vi "GpuMat RowRange.vi"(8 "error in (no error)":errorcluster, 9 "EndRow":i32, 10 "StartRow":i32, 11 "Src in":refnum<class "GpuMat.lvclass">) -> (0 "error out":errorcluster, 2 "Clone out":refnum<class "GpuMat.lvclass">, 3 "Src out":refnum<class "GpuMat.lvclass">)   [LabVIEW 2020, in "OpenLvVision_OpenCv.lvlib" / "Cuda.lvlib" / "GpuMat.lvclass"]
doc: "returns a new GpuMat header for the specified row span"
uses:
  GpuMat.lvclass
  C:/Users/lukas/Documents/OpenLvVision_OpenCv/SourceCode/LabView/OpenLvVision_OpenCv/_LvHelpers/EdvrObject/EdvrObject.lvclass
  _LvHelpers/EdvrObject/EdvrObject.lvclass/EdvrObject.ctl
  _LvHelpers/EdvrObject/TypeDef/Edvr.ctl
  OpenLvVision_OpenCv.lvlib
  <vilib>/Utility/error.llb/Error Cluster From Error Code.vi
  <vilib>/ErrorRing/Error Ring.xnode
  _LvHelpers/EdvrObject/EdvrObject.lvclass
  Dlls/OlvOpenCvWrapper.dll
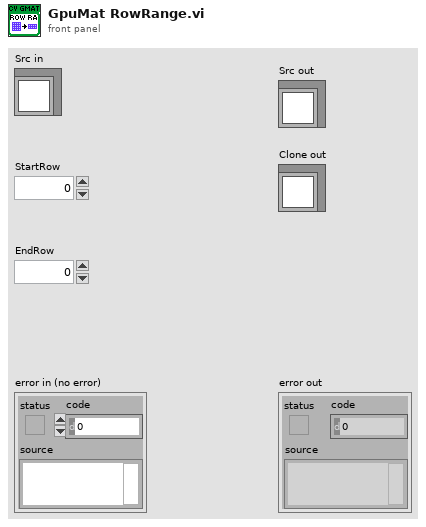
[diagram p1: front panel]
types:
  T1 = typedef "OpenLvVision_OpenCv.lvlib/EdvrObject.lvclass/Edvr.ctl" = refnum<data-value>
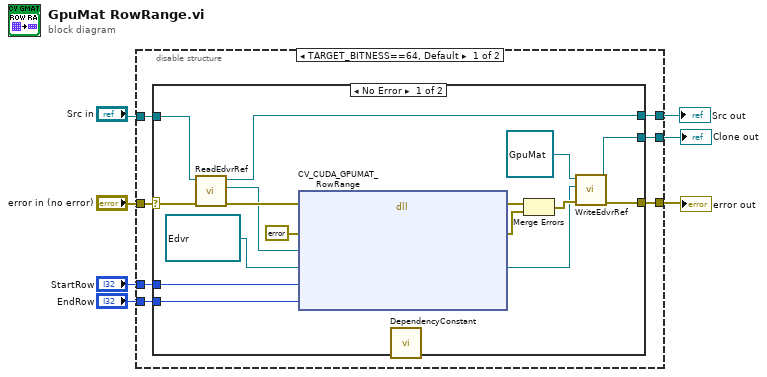
[diagram p0: block diagram]
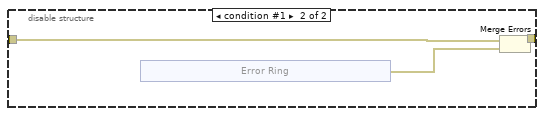
[diagram p3: hidden frame]
diagram:
  n1 = disable-structure shown="TARGET_BITNESS==64, Default" {
    disable-tunnel: "error in (no error)" -> [w14 w34]
    disable-tunnel: [w13 w35] -> w7
    disable-tunnel: "Src in" -> [w12 _]
    disable-tunnel: [w11 _] -> w4
    disable-tunnel: [w10 _] -> w3
    disable-tunnel: "StartRow" -> [w9 _]
    disable-tunnel: "EndRow" -> [w8 _]
    frame condition #0 (active) {
      n2 = case shown="No Error" w14 {
        selector: w14 -> [w23 w32]
        tunnel: [w21 w32] -> w13
        tunnel: w12 -> [w25 w31]
        tunnel: [w24 w31] -> w11
        tunnel: [w19 _] -> w10
        tunnel: w9 -> [w16 _]
        tunnel: w8 -> [w15 _]
        frame No Error {
          n3 = call "ReadEdvrRef.vi"("error in (no error)"=w23, "EdvrObject in"=w25) -> ("error out"=w27:errorcluster, "Edvr"=w26:T1, "EdvrObject out"=w24:refnum<class "GpuMat.lvclass">)  [unwired: 7 in]
          n4 = dll-call lib="C:/Users/lukas/Documents/OpenLvVision_OpenCv/SourceCode/LabView/OpenLvVision_OpenCv/Dlls/OlvOpenCvWrapper.dll" fn="CV_CUDA_GPUMAT_RowRange"(error in=w27, "Error"=errorcluster {"status"=FALSE, "code"=0, "source"=""} ("error out"), "srcRef"=w26, "dstRef"=T1 refnum ("Edvr"), "startCol"=w16, "endCol"=w15) -> (error out=w30:errorcluster, "Error"=w29:errorcluster, "dstRef"=w18:T1)  [unwired: 6 in, 1 out]
          n5 = call "DependencyConstant.vi"() -> ()  [unwired: 12 in]
          n6 = Merge Errors(w30, w29) -> (w22:errorcluster)
          n7 = call "WriteEdvrRef.vi"("error in (no error)"=w22, "Edvr"=w18, "EdvrObject in"=refnum<class "GpuMat.lvclass"> refnum ("Dst out")) -> ("error out"=w21:errorcluster, "EdvrObject out"=w19:refnum<class "GpuMat.lvclass">)  [unwired: 7 in]
        }
        frame Error {
        }
      }
    }
    frame condition #1 {
      n8 = xnode "Error Ring"() -> ("error out"=w33:errorcluster)
      n9 = Merge Errors(w34, w33) -> (w35:errorcluster)
    }
  }
  "error out" <- w7
  "Clone out" <- w3
  "Src out" <- w4
